vi "test tool automatic error handling.vi"(8 "error in (no error)":errorcluster) -> (0 "error out":errorcluster, 3 "body":string)   [LabVIEW 2020, in "MCP Server tests.lvlib"]
doc: "fake_tool_unwired_error has automatic error handling enabled and leaves the error of its JSON parse unwired. Called with json = \"not json\", once plainly and once streamed, it must be answered (a result, no JSON-RPC error) and the server must answer the next request. Before the fix LabVIEW opened its modal error dialog for the tool VI and the server stopped answering."
uses:
  MCP Server tests.lvlib
  <vilib>/JDP Science/JSONtext/Next JSON Value.vi
  <vilib>/JDP Science/JSONtext/String Subset.vi
  <vilib>/JDP Science/JSONtext/Parsing/Advance past next JSON Value (inlined COPY).vi
  <vilib>/JDP Science/JSONtext/Parsing/Advance past whitespace.vi
  <vilib>/JDP Science/JSONtext/Parsing/Advance past String.vi
  <vilib>/JDP Science/JSONtext/Parsing/Advance past Number.vi
  <vilib>/JDP Science/JSONtext/Parsing/Advance past Line Ending.vi
  <vilib>/JDP Science/JSONtext/Parsing/Parse Full Path or Item Name.vi
  <vilib>/JDP Science/JSONtext/Parsing/Advance past Array.vi
  <vilib>/JDP Science/JSONtext/Parsing/Advance past Object.vi
  <vilib>/JDP Science/JSONtext/support/Error Cluster From Code.vi
  <vilib>/JDP Science/JSONtext/Offset/Find Item Locations by Path.vi
  <vilib>/addons/_JKI Toolkits/Caraya/classes/Test/Test.lvclass
  <vilib>/addons/_JKI Toolkits/Caraya/classes/Assert/Assert.lvclass
  <vilib>/JDP Science/JSONtext/JSONtext.lvlib
panel:
  out "lookup error":errorcluster
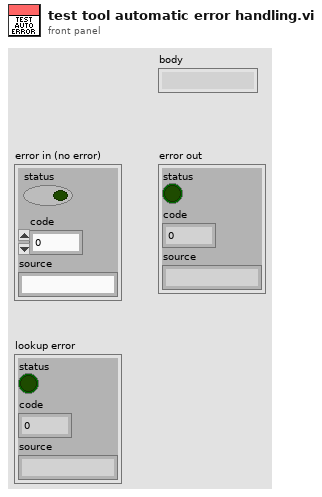
[diagram p1: front panel]
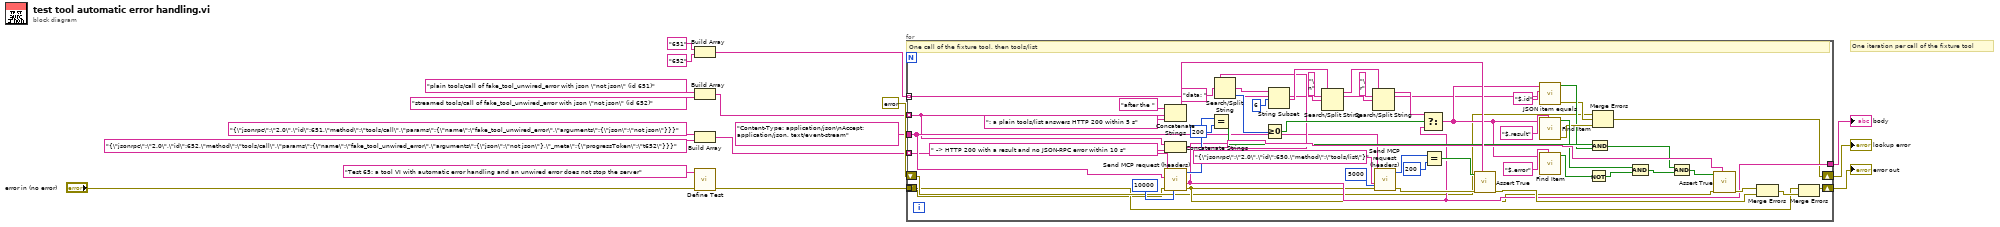
[diagram p0: block diagram]
diagram:
  # "One iteration per call of the fixture tool"
  n1 = Build Array("651" ("id 651"), "652" ("id 652")) -> (w12:string[])
  n2 = Build Array("plain tools/call of fake_tool_unwired_error with json \"not json\" (id 651)" ("label 651"), "streamed tools/call of fake_tool_unwired_error with json \"not json\" (id 652)" ("label 652")) -> (w15:string[])
  n3 = Build Array("{\"jsonrpc\":\"2.0\",\"id\":651,\"method\":\"tools/call\",\"params\":{\"name\":\"fake_tool_unwired_error\",\"arguments\":{\"json\":\"not json\"}}}" ("request 651"), "{\"jsonrpc\":\"2.0\",\"id\":652,\"method\":\"tools/call\",\"params\":{\"name\":\"fake_tool_unwired_error\",\"arguments\":{\"json\":\"not json\"},\"_meta\":{\"progressToken\":\"t652\"}}}" ("request 652")) -> (w9:string[])
  n4 = call <vilib>:"Define Test.vi"("error in (no error)"="error in (no error)", "Label (VI Title)"="Test 65: a tool VI with automatic error handling and an unwired error does not stop the server") -> ("error out"=w6:errorcluster)  [unwired: 8 in, 1 out]
  n5 = for {
    tunnel: "Content-Type: application/json\nAccept: application/json, text/event-stream" ("request headers") -> [w21]
    shift-right: [w27] -> w3
    shift-left: errorcluster {"status"=FALSE, "code"=0, "source"=""} ("no lookup error") -> [w26]
    tunnel: w9 -> [w18] mode=indexing
    tunnel: w12 -> [w19] mode=indexing
    tunnel: w15 -> [w20] mode=indexing
    tunnel: w6 -> [w22]
    shift-right: [w23] -> w4
    shift-left: w6 -> [w24]
    tunnel: [w30] -> w2
    # "One call of the fixture tool, then tools/list"
    n6 = Concatenate Strings("after the " ("after"), w20, ": a plain tools/list answers HTTP 200 within 5 s" ("text 2")) -> (w68:string)
    n7 = Concatenate Strings(w20, " -> HTTP 200 with a result and no JSON-RPC error within 10 s" ("text 1")) -> (w58:string)
    n8 = call "Send MCP request (headers).vi"("timeout (10000)"=10000 ("timeout"), "error in (no error)"=w22, "request"=w18, "request headers"=w21) -> ("error out"=w29:errorcluster, "response"=w30:string, "status code"=w31:i32)  [unwired: 4 in, 1 out]
    n9 = Equal?(x=w31, y=200 ("expected 200")) -> (x = y?=w53:bool)
    n10 = Search/Split String(string=w30, search string/char (-)="data: " ("data marker")) -> (match + rest of string=w34:string, offset of match=w33:i32)  [unwired: 1 in, 1 out]
    n11 = Greater Or Equal To 0?(x=w33) -> (x >= 0?=w41:bool)
    n12 = String Subset(string=w34, offset (0)=6 ("after data:")) -> (substring=w36:string)  [unwired: 1 in]
    n13 = Search/Split String(string=w36, search string/char (-)="\n" ("line feed")) -> (substring before match=w38:string)  [unwired: 1 in, 2 out]
    n14 = Search/Split String(string=w38, search string/char (-)="\r" ("carriage return")) -> (substring before match=w40:string)  [unwired: 1 in, 2 out]
    n15 = call "Send MCP request (headers).vi"("timeout (10000)"=5000 ("5 s"), "error in (no error)"=w29, "request"="{\"jsonrpc\":\"2.0\",\"id\":650,\"method\":\"tools/list\"}" ("tools/list"), "request headers"=w21) -> ("error out"=w62:errorcluster, "status code"=w63:i32)  [unwired: 4 in, 2 out]
    n16 = Select(t=w40, s=w41, f=w30) -> (s? t:f=w42:string)
    n17 = Equal?(x=w63, y=200 ("expected 200")) -> (x = y?=w65:bool)
    n18 = call <vilib>:"Assert True.vi"("Label"=w68, "error in (no error)"=w62, "True?"=w65) -> ("error out"=w69:errorcluster)  [unwired: 7 in, 1 out]
    n19 = call "JSON item equals.vi"("expected"=w19, "path"="$.id" ("id path"), "JSON"=w42) -> ("error out"=w44:errorcluster, "equal?"=w45:bool)  [unwired: 6 in, 1 out]
    n20 = call <vilib>:"Find Item.vi"("$Path or Item Name"="$.result" ("result path"), "JSON"=w42) -> ("error out"=w47:errorcluster, "Found"=w48:bool)  [unwired: 6 in, 2 out]
    n21 = call <vilib>:"Find Item.vi"("$Path or Item Name"="$.error" ("error path"), "JSON"=w42) -> ("Found"=w50:bool)  [unwired: 6 in, 3 out]
    n22 = Not(x=w50) -> (.not. x?=w51:bool)
    n23 = And(x=w53, y=w45) -> (x .and. y?=w54:bool)
    n24 = Merge Errors(w26, w44, w47) -> (w27:errorcluster)
    n25 = And(x=w48, y=w51) -> (x .and. y?=w55:bool)
    n26 = And(x=w54, y=w55) -> (x .and. y?=w56:bool)
    n27 = call <vilib>:"Assert True.vi"("Label"=w58, "error in (no error)"=w29, "True?"=w56) -> ("error out"=w59:errorcluster)  [unwired: 7 in, 1 out]
    n28 = Merge Errors(w59, w69) -> (w25:errorcluster)
    n29 = Merge Errors(w24, w25) -> (w23:errorcluster)
  }
  "body" <- w2
  "lookup error" <- w3
  "error out" <- w4
